vi "Playground.vi"(11 "Inset":refnum<class "Inset.lvclass">) -> ()   [LabVIEW 2019, in "Inset.lvclass"]
uses:
  Inset.lvclass
  BigMAQ/BigMAQ.lvclass
  Parse/ParseXML/ParseSVG.lvclass
  Parse/ParseVectorFile/ParseVectorFile.lvclass
  Parse/ParseXML/Image.ctl
  Parse/EditSVG/EditSVG.lvclass
  <vilib>/LabVIEW Open Source Project/OpenURI/openURI.lvlib
  Parse/Image/SVGImage.lvclass
panel:
  out "Edited XML":string
  out "BGD Size":dbl
  out "Y Offset 2":string
  out "ScanSize 2":string
  out "BGD Y Offset":dbl
  out "BGD X Offset":dbl
  out "Inset X Offset":dbl
  out "Inset Y Offset":dbl
  out "Inset Size":dbl
  out "SVGImage.lvclass":refnum<class "SVGImage.lvclass">
  out "ScanSize":string
  out "Y Offset":string
  in  "Inkscape Path":path
  in  "Background Path":path=path "C:/Users/Albro/Documents/GitHub/AFM-Lithography/test files/Inset Test Files/R_tMLG_Au0003.ibw"
  in  "Inset Path":path=path "C:/Users/Albro/Documents/GitHub/AFM-Lithography/test files/Inset Test Files/R_tMLG_Au0004.ibw"
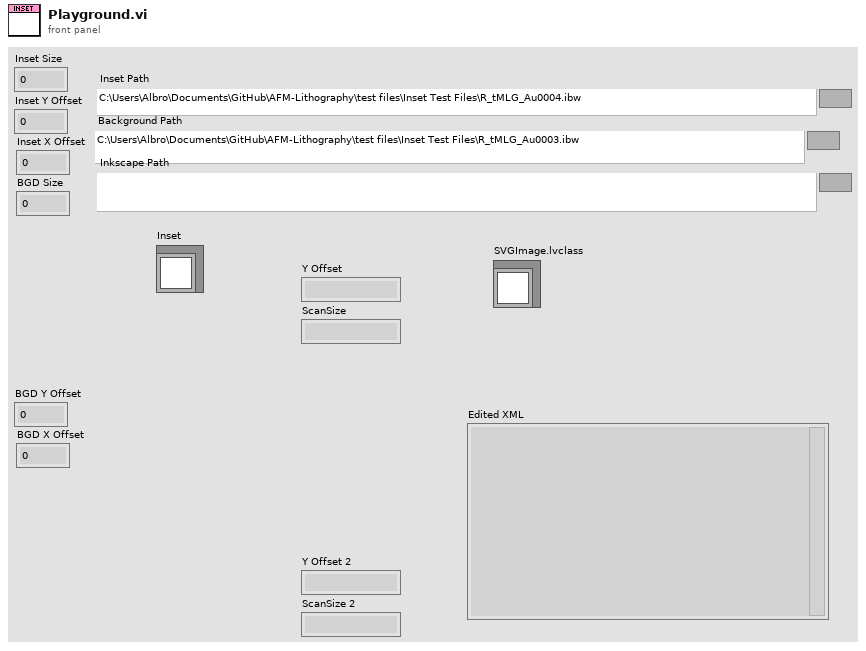
[diagram p1: front panel]
types:
  T1 = cluster{"Inkscape":path, "Background":path, "Inset":path}
  T2 = typedef "ParseSVG.lvclass/Image.ctl" = cluster{"x":string, "y":string, "width":string, "height":string, "xlink:href":string, "id":string, "transform":string}
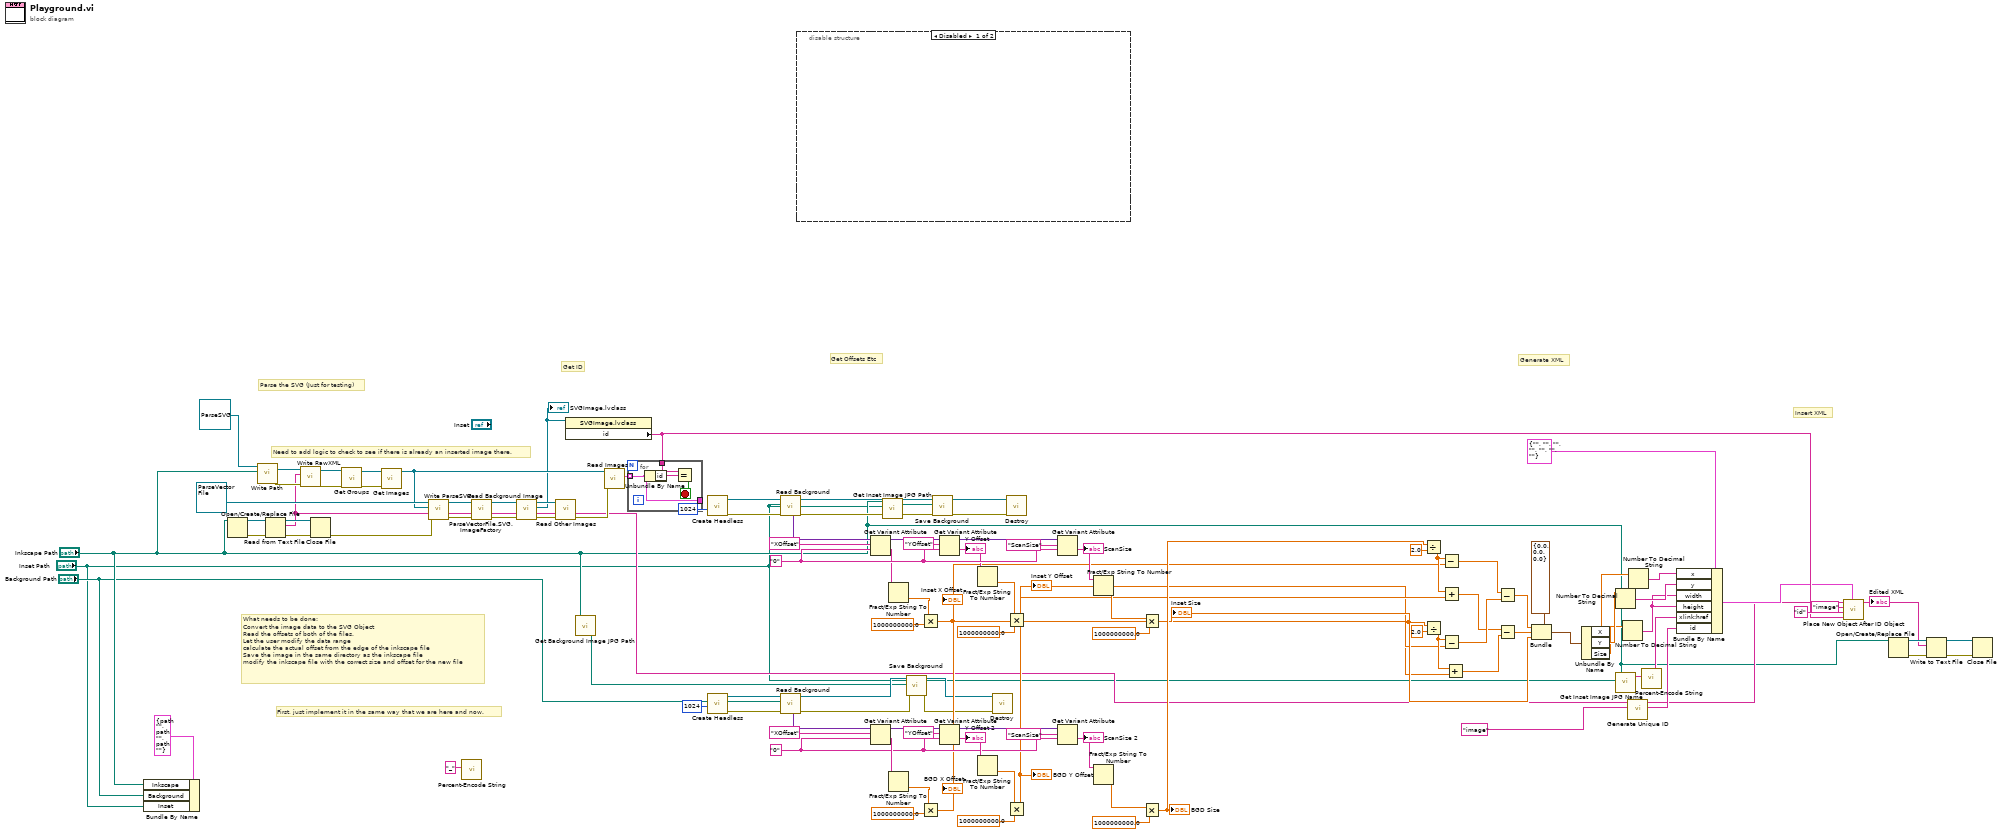
[diagram p0: block diagram]
diagram:
  w62 = "0"
  w110 = "0"
  # "First, just implement it in the same way that we are here and now."
  # "Parse the SVG (Just for testing)"
  # "Insert XML"
  # "Generate XML"
  # "Get Offsets Etc"
  # "Get ID"
  # "Need to add logic to check to see if there is already an inserted image there."
  # "What needs to be done:\nConvert the image data to the SVG Object\nRead the offsets of both of the files.\nLet the user modify the data range\ncalculate the actual offset from the edge of the inkscape file\nSave the image in the same directory as the inkscape file\nmodify the inkscape file with the correct size and offset for the new file"
  n1 = Bundle By Name(cluster=T1 {"Inkscape"=path "", "Background"=path "", "Inset"=path ""} ("Paths"), "Inkscape"="Inkscape Path", "Background"="Background Path", "Inset"="Inset Path") -> ()  [unwired: 1 out]
  n2 = Open/Create/Replace File(file path (use dialog)="Inkscape Path") -> (refnum out=w99:refnum<file>, error out=w97:errorcluster)  [unwired: 5 in, 1 out]
  n3 = call-dynamic "Write Path.vi"("Path"="Inkscape Path", "ParseSVG in"=refnum<class "ParseSVG.lvclass"> refnum) -> ("error out"=w107:errorcluster, "ParseSVG out"=w108:refnum<class "ParseSVG.lvclass">)  [unwired: 8 in]
  n4 = Read from Text File(file (use dialog)=w99, error in=w97) -> (refnum out=w98:refnum<file>, text=w13:string, error out=w96:errorcluster)  [unwired: 2 in, 1 out]
  n5 = call "Write RawXML.vi"("error in (no error)"=w107, "RawXML"=w13, "ParseSVG.lvclass"=w108) -> ("error out"=w105:errorcluster, "ParseSVG.lvclass 2"=w106:refnum<class "ParseSVG.lvclass">)  [unwired: 7 in]
  n6 = Close File(refnum=w98, error in=w96) -> (error out=w95:errorcluster)  [unwired: 1 out]
  n7 = call "Get Groups.vi"("error in (no error)"=w105, "ParseSVG in"=w106) -> ("error out"=w103:errorcluster, "ParseSVG out"=w104:refnum<class "ParseSVG.lvclass">)  [unwired: 8 in]
  n8 = call "Get Images.vi"("error in (no error)"=w103, "ParseSVG in"=w104) -> ("ParseSVG out"=w89:refnum<class "ParseSVG.lvclass">)  [unwired: 8 in, 1 out]
  n9 = call-dynamic "Write ParseSVG.vi"("error in (no error)"=w95, "ParseSVG.lvclass"=w89, "ParseVectorFile in"=refnum<class "ParseVectorFile.lvclass"> refnum ("ParseVectorFile.lvclass")) -> ("error out"=w100:errorcluster, "ParseVectorFile out"=w101:refnum<class "ParseVectorFile.lvclass">)  [unwired: 7 in]
  n10 = call <vilib>:"Percent-Encode String.vi"("String"="_") -> ()  [unwired: 10 in, 1 out]
  n11 = call "ParseVectorFile.SVG.ImageFactory.vi"("error in (no error)"=w100, "ParseVectorFile in"=w101) -> ("error out"=w93:errorcluster, "ParseVectorFile out"=w94:refnum<class "ParseVectorFile.lvclass">)  [unwired: 8 in]
  n12 = call-dynamic "Read Background Image.vi"("error in (no error)"=w93, "ParseVectorFile in"=w94) -> ("error out"=w91:errorcluster, "SVGImage.lvclass"=w1:refnum<class "SVGImage.lvclass">, "ParseVectorFile out"=w92:refnum<class "ParseVectorFile.lvclass">)  [unwired: 7 in]
  "SVGImage.lvclass" <- w1
  n13 = call-dynamic "Read Other Images.vi"("error in (no error)"=w91, "ParseVectorFile in"=w92) -> ("error out"=w90:errorcluster)  [unwired: 7 in, 2 out]
  n14 = property class="SVGImage.lvclass"(reference=w1) -> ("id"=w22:string)  [unwired: 1 in, 2 out]
  n15 = call "Get Background Image JPG Path.vi"("Inkscape Path"="Inkscape Path") -> ("Background JPG Path"=w9:path)  [unwired: 2 in]
  n16 = call "Read Images.vi"("error in (no error)"=w90, "ParseSVG in"=w89) -> ("Images"=w88:T2[])  [unwired: 7 in, 2 out]
  n17 = for {
    tunnel: w88 -> [w116] mode=indexing
    tunnel: w22 -> [w118]
    tunnel: [w116] -> _
    stop <- w117 stop-if-true
    n18 = Unbundle By Name(w116) -> ("id"=w119:string)
    n19 = Equal?(x=w118, y=w119) -> (x = y?=w117:bool)
  }
  n20 = call "Create Headless.vi"("Resolution"=1024) -> ("error out"=w85:errorcluster, "BigMAQ out"=w86:refnum<class "BigMAQ.lvclass">)  [unwired: 9 in]
  n21 = call "Create Headless.vi"("Resolution"=1024) -> ("error out"=w73:errorcluster, "BigMAQ out"=w74:refnum<class "BigMAQ.lvclass">)  [unwired: 9 in]
  n22 = call "Read Background.vi"("error in (no error)"=w85, "Path"="Inset Path", "BigMAQ in"=w86) -> ("error out"=w52:errorcluster, "BigMAQ out"=w55:refnum<class "BigMAQ.lvclass">, "Metadata"=w84:variant)  [unwired: 6 in]
  n23 = call "Read Background.vi"("error in (no error)"=w73, "Path"="Background Path", "BigMAQ in"=w74) -> ("error out"=w10:errorcluster, "BigMAQ out"=w12:refnum<class "BigMAQ.lvclass">, "Metadata"=w56:variant)  [unwired: 6 in]
  n24 = disable-structure shown="Disabled" {
    frame Disabled {
    }
    frame Enabled {
    }
  }
  n25 = Get Variant Attribute(Variant=w84, name="XOffset", default value (empty Variant)=w110) -> (duplicate Variant=w114:variant, value=w81:string)  [unwired: 1 in, 2 out]
  n26 = Get Variant Attribute(Variant=w56, name="XOffset", default value (empty Variant)=w62) -> (duplicate Variant=w58:variant, value=w65:string)  [unwired: 1 in, 2 out]
  n27 = call "Get Inset Image JPG Path.vi"("Inset Data Path"="Inset Path", "Inkscape Path"="Inkscape Path") -> ("Inset JPG Path"=w53:path)  [unwired: 3 in]
  n28 = Fract/Exp String To Number(string=w81) -> (number=w80:dbl)  [unwired: 3 in, 1 out]
  n29 = Fract/Exp String To Number(string=w65) -> (number=w66:dbl)  [unwired: 3 in, 1 out]
  n30 = call "Save Background.vi"("error in"=w10, "File Path"=w9, "BigMAQ in"=w12) -> ("error out"=w4:errorcluster, "BigMAQ out"=w11:refnum<class "BigMAQ.lvclass">)  [unwired: 7 in]
  n31 = Multiply(x=w80, y=1000000000.0) -> (x*y=w37:dbl)
  "Inset X Offset" <- w37
  n32 = Multiply(x=w66, y=1000000000.0) -> (x*y=w40:dbl)
  "BGD X Offset" <- w40
  n33 = call "Save Background.vi"("error in"=w52, "File Path"=w53, "BigMAQ in"=w55) -> ("error out"=w5:errorcluster, "BigMAQ out"=w54:refnum<class "BigMAQ.lvclass">)  [unwired: 7 in]
  n34 = Get Variant Attribute(Variant=w114, name="YOffset", default value (empty Variant)=w110) -> (duplicate Variant=w112:variant, value=w82:string)  [unwired: 1 in, 2 out]
  "Y Offset" <- w82
  n35 = Get Variant Attribute(Variant=w58, name="YOffset", default value (empty Variant)=w62) -> (duplicate Variant=w60:variant, value=w64:string)  [unwired: 1 in, 2 out]
  "Y Offset 2" <- w64
  n36 = Fract/Exp String To Number(string=w82) -> (number=w77:dbl)  [unwired: 3 in, 1 out]
  n37 = Fract/Exp String To Number(string=w64) -> (number=w69:dbl)  [unwired: 3 in, 1 out]
  n38 = call "Destroy.vi"("error in"=w4, "BigMAQ in"=w11) -> ()  [unwired: 8 in, 2 out]
  n39 = call "Destroy.vi"("error in"=w5, "BigMAQ in"=w54) -> ()  [unwired: 8 in, 2 out]
  n40 = Multiply(x=w77, y=1000000000.0) -> (x*y=w36:dbl)
  "Inset Y Offset" <- w36
  n41 = Multiply(x=w69, y=1000000000.0) -> (x*y=w39:dbl)
  "BGD Y Offset" <- w39
  n42 = Get Variant Attribute(Variant=w112, name="ScanSize", default value (empty Variant)=w110) -> (value=w83:string)  [unwired: 1 in, 3 out]
  "ScanSize" <- w83
  n43 = Get Variant Attribute(Variant=w60, name="ScanSize", default value (empty Variant)=w62) -> (value=w63:string)  [unwired: 1 in, 3 out]
  "ScanSize 2" <- w63
  n44 = Fract/Exp String To Number(string=w83) -> (number=w75:dbl)  [unwired: 3 in, 1 out]
  n45 = Fract/Exp String To Number(string=w63) -> (number=w71:dbl)  [unwired: 3 in, 1 out]
  n46 = Multiply(x=w75, y=1000000000.0) -> (x*y=w38:dbl)
  "Inset Size" <- w38
  n47 = Multiply(x=w71, y=1000000000.0) -> (x*y=w41:dbl)
  "BGD Size" <- w41
  n48 = Divide(x=w41, y=2.0) -> (x/y=w50:dbl)
  n49 = Divide(x=w38, y=2.0) -> (x/y=w49:dbl)
  n50 = Subtract(x=w50, y=w40) -> (x-y=w47:dbl)
  n51 = Add(x=w50, y=w39) -> (x+y=w45:dbl)
  n52 = Subtract(x=w49, y=w37) -> (x-y=w46:dbl)
  n53 = Add(x=w49, y=w36) -> (x+y=w44:dbl)
  n54 = Subtract(x=w47, y=w46) -> (x-y=w42:dbl)
  n55 = Subtract(x=w45, y=w44) -> (x-y=w43:dbl)
  n56 = Bundle(cluster=cluster{"X":dbl, "Y":dbl, "Size":dbl} {"X"=0.0, "Y"=0.0, "Size"=0.0}, "X"=w42, "Y"=w43, "Size"=w38) -> (w33:cluster{"X":dbl, "Y":dbl, "Size":dbl})
  n57 = Unbundle By Name(w33) -> ("X"=w32:dbl, "Y"=w30:dbl, "Size"=w28:dbl)
  n58 = Number To Decimal String(number=w30) -> (decimal integer string=w29:string)  [unwired: 1 in]
  n59 = call "Get Inset Image JPG Name.vi"("Inset Data Path"="Inset Path", "Inkscape Path"="Inkscape Path") -> ("Inset JPG Name"=w20:string)  [unwired: 3 in]
  n60 = Number To Decimal String(number=w28) -> (decimal integer string=w27:string)  [unwired: 1 in]
  n61 = call "Generate Unique ID.vi"("Basename"="image", "XML String"=w13) -> ("Unique ID"=w26:string)  [unwired: 9 in]
  n62 = Number To Decimal String(number=w32) -> (decimal integer string=w31:string)  [unwired: 1 in]
  n63 = call <vilib>:"Percent-Encode String.vi"("String"=w20) -> ("Pct-Encoded String"=w19:string)  [unwired: 10 in]
  n64 = Bundle By Name(cluster=T2 {"x"="", "y"="", "width"="", "height"="", "xlink:href"="", "id"="", "transform"=""} ("image"), "x"=w31, "y"=w29, "width"=w27, "height"=w27, "xlink:href"=w19, "id"=w26) -> (w21:T2)
  n65 = call "Place New Object After ID Object.vi"("Named Cluster"=w21, "Identifying Attribute Value"=w22, "Identifying Attribute Type"="id", "Element Type"="image", "XML String"=w13) -> ("Edited XML"=w14:string)  [unwired: 6 in]
  "Edited XML" <- w14
  n66 = Open/Create/Replace File(file path (use dialog)="Inkscape Path") -> (refnum out=w16:refnum<file>, error out=w18:errorcluster)  [unwired: 5 in, 1 out]
  n67 = Write to Text File(file (use dialog)=w16, text=w14, error in=w18) -> (refnum out=w15:refnum<file>, error out=w17:errorcluster)  [unwired: 1 in, 1 out]
  n68 = Close File(refnum=w15, error in=w17) -> ()  [unwired: 2 out]
